vi "Dispatch Get Metadata Async.vi"(8 "error in (no error)":errorcluster, 10 "measurement plugin service in":refnum<class "Measurement Plugin Service.lvclass">, 11 "gRPC ID in":T1) -> (0 "error out":errorcluster)   [LabVIEW 2021, in "NI Measurement Plug-In SDK.lvlib" / "Measurement Service V2.lvclass"]
uses:
  Measurement Service V2.lvclass
  <vilib>/gRPC/LabVIEW gRPC Library/Shared/grpcId.ctl
  Measurement Plugin Service/Measurement Plugin Service.lvclass
  Handle Get Metadata RPC.vi
  IMeasurement Service/IMeasurement Service.lvclass
  <vilib>/gRPC/LabVIEW gRPC Library/grpc-lvsupport-release.lvlib
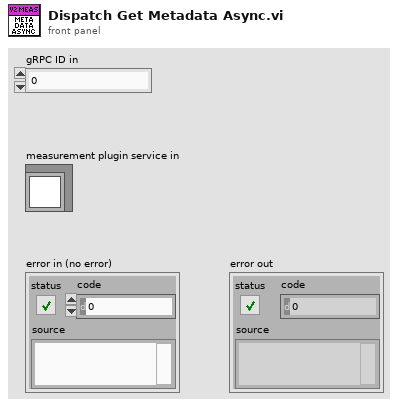
[diagram p1: front panel]
types:
  T1 = typedef "grpc-lvsupport-release.lvlib/grpcId.ctl" = u64
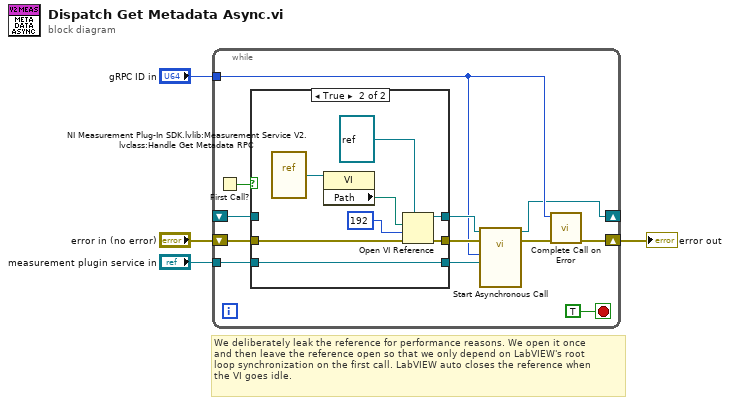
[diagram p0: block diagram]
diagram:
  # "We deliberately leak the reference for performance reasons. We open it once\nand then leave the reference open so that we only depend on LabVIEW's root\nloop synchronization on the first call. LabVIEW auto closes the reference when\nthe VI goes idle."
  n1 = while {
    tunnel: "gRPC ID in" -> [w12]
    tunnel: "measurement plugin service in" -> [w10]
    shift-right: [w13] -> w3
    shift-left: "error in (no error)" -> [w14]
    shift-right: [w5] -> _
    shift-left: _ -> [w6]
    stop <- TRUE stop-if-true
    n2 = First Call?() -> (First Call?: T/F=w11:bool)
    n3 = case shown="True" w11 {
      tunnel: [w17 w25] -> w16
      tunnel: [w18 w24] -> w15
      tunnel: w14 -> [w18 w23]
      tunnel: w10 -> [w19 w20]
      tunnel: [w19 w20] -> w9
      tunnel: w6 -> [w17 _]
      frame False {
      }
      frame True {
        n4 = vi-ref "NI Measurement Plug-In SDK.lvlib:Measurement Service V2.lvclass:Handle Get Metadata RPC.vi"() -> (w22:refnum<vi>)
        n5 = property class="VI"(reference=w22) -> ("Path"=w21:path)  [unwired: 1 in, 2 out]
        n6 = Open VI Reference(type specifier VI Refnum (for type only)=refnum<vi> refnum, vi path=w21, options=192, error in (no error)=w23) -> (vi reference=w25:refnum<vi>, error out=w24:errorcluster)  [unwired: 2 in]
      }
    }
    n7 = call-by-ref "Start Asynchronous Call"(reference=w16, error in=w15, "measurement plugin service in"=w9, "gRPC ID"=w12) -> (reference out=w5:refnum<vi>, error out=w8:errorcluster)  [unwired: 10 in]
    n8 = call "Complete Call on Error.vi"("error in"=w8, "gRPC ID in"=w12) -> ("error out"=w13:errorcluster)  [unwired: 9 in]
  }
  "error out" <- w3
